vi "GetHeader.vi"(8 "error in (no error)":errorcluster, 10 "Name":string, 11 "Headers In":variant) -> (0 "error out":errorcluster, 1 "Found?":bool, 2 "Data":string, 3 "Headers Out":variant)   [LabVIEW 2021, in "LV WebSockets.lvlib"]
doc: "Retrieves a named header from the received HTTP handshaking data.\nWebSockets 1.6.0.22\nSam Sharp - MediaMongrels Ltd\nCopyright (c) 2016, MediaMongrels Ltd"
uses:
  LV WebSockets.lvlib
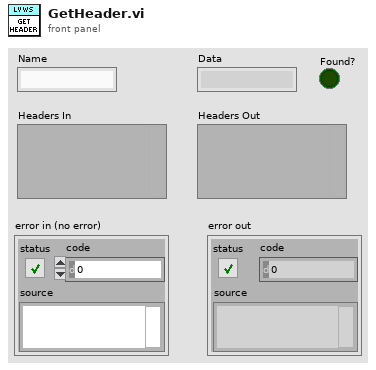
[diagram p1: front panel]
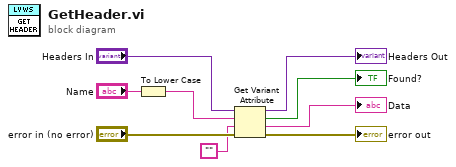
[diagram p0: block diagram]
diagram:
  n1 = To Lower Case(string="Name") -> (all lower case string=w1:string)
  n2 = Get Variant Attribute(Variant="Headers In", name=w1, default value (empty Variant)="", error in="error in (no error)") -> (duplicate Variant=→"Headers Out":variant, found=→"Found?":bool, value=→"Data":string, error out=→"error out":errorcluster)
